vi "Work_2 Cooker Module.vi"() -> ()   [LabVIEW 2026]
panel:
  in  "number":i32
  in  "Burgers":bool
  in  "Meal":bool
  in  "Stop":bool
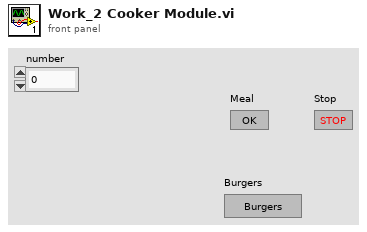
[diagram p1: front panel]
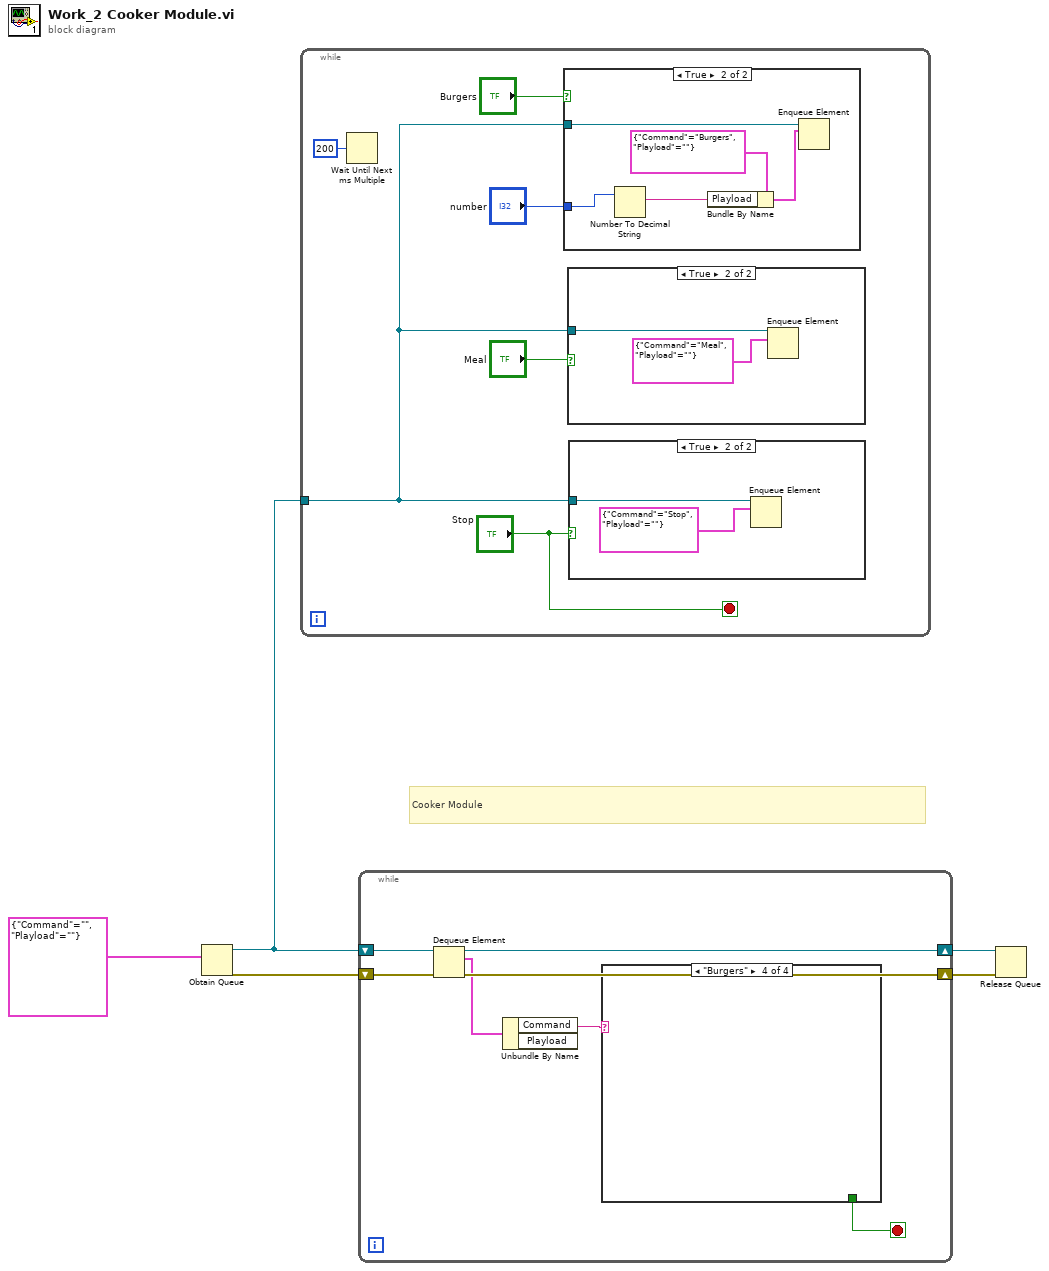
[diagram p0: block diagram]
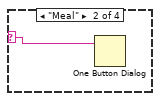
[diagram p6: hidden frame]
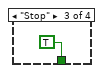
[diagram p7: hidden frame]
diagram:
  # "Cooker Module"
  n1 = Obtain Queue(element data type=cluster{"Command":string, "Playload":string} {"Command"="", "Playload"=""}) -> (queue out=w2:refnum<queue>, error out=w4:errorcluster)  [unwired: 4 in, 1 out]
  n2 = while {
    tunnel: w2 -> [w7]
    stop <- "Stop" stop-if-true
    n3 = Wait Until Next ms Multiple(millisecond multiple=u32 200) -> ()  [unwired: 1 out]
    n4 = case shown="True" "Burgers" {
      tunnel: w7 -> [_ w16]
      tunnel: "number" -> [_ w14]
      frame False {
      }
      frame True {
        n5 = Number To Decimal String(number=w14) -> (decimal integer string=w15:string)  [unwired: 1 in]
        n6 = Bundle By Name(cluster=cluster{"Command":string, "Playload":string} {"Command"="Burgers", "Playload"=""} ("element"), "Playload"=w15) -> (w12:cluster{"Command":string, "Playload":string})
        n7 = Enqueue Element(queue=w16, element=w12) -> ()  [unwired: 2 in, 3 out]
      }
    }
    n8 = case shown="True" "Meal" {
      tunnel: w7 -> [_ w18]
      frame False {
      }
      frame True {
        n9 = Enqueue Element(queue=w18, element=cluster{"Command":string, "Playload":string} {"Command"="Meal", "Playload"=""}) -> ()  [unwired: 2 in, 3 out]
      }
    }
    n10 = case shown="True" "Stop" {
      tunnel: w7 -> [_ w20]
      frame False {
      }
      frame True {
        n11 = Enqueue Element(queue=w20, element=cluster{"Command":string, "Playload":string} {"Command"="Stop", "Playload"=""}) -> ()  [unwired: 2 in, 3 out]
      }
    }
  }
  n12 = while {
    shift-right: [w25] -> w3
    shift-left: w4 -> [w26]
    shift-right: [w27] -> w5
    shift-left: w2 -> [w24]
    stop <- w21 stop-if-true
    n13 = Dequeue Element(queue=w24, error in (no error)=w26) -> (queue out=w27:refnum<queue>, element=w23:cluster{"Command":string, "Playload":string}, error out=w25:errorcluster)  [unwired: 1 in, 1 out]
    n14 = Unbundle By Name(w23) -> ("Command"=w22:string)  [unwired: 1 out]
    n15 = case shown="\"Burgers\"" w22 {
      selector: w22 -> [_ w28 _ _]
      tunnel: [_ _ TRUE _] -> w21
      frame Default {
      }
      frame "Meal" {
        n16 = One Button Dialog(message=w28) -> ()  [unwired: 1 in, 1 out]
      }
      frame "Stop" {
      }
      frame "Burgers" {
      }
    }
  }
  n17 = Release Queue(queue=w5, error in (no error)=w3) -> ()  [unwired: 1 in, 3 out]
